vi "Save TS DAC Configuration.vi"(8 "error in":errorcluster, 11 "Generic Test Stand in":refnum<class "Generic Test Stand.lvclass">) -> (0 "error out":errorcluster, 3 "Generic Test Stand out":refnum<class "Generic Test Stand.lvclass">)   [LabVIEW 2019, in "Generic Test Stand.lvclass"]
uses:
  Generic Test Stand.lvclass
  Generic Test Stand.lvclass/Generic Test Stand.ctl
  DAC/DAC.lvclass
  <vilib>/Utility/config.llb/NI_LVConfig.lvlib
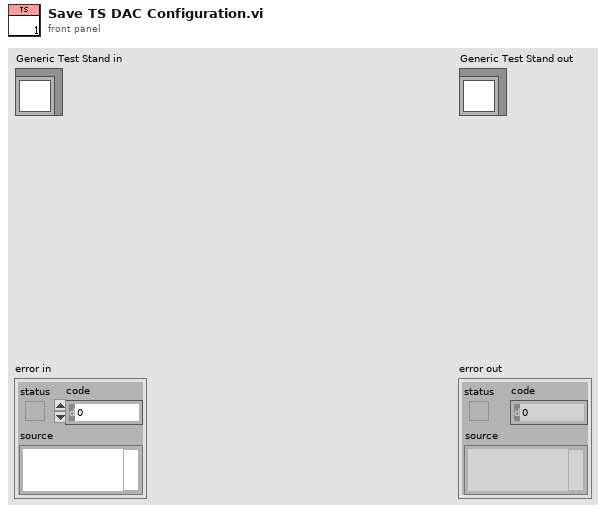
[diagram p1: front panel]
types:
  T1 = typedef "NI_LVConfig.lvlib/Config Data RefNum.ctl" = refnum<k1>
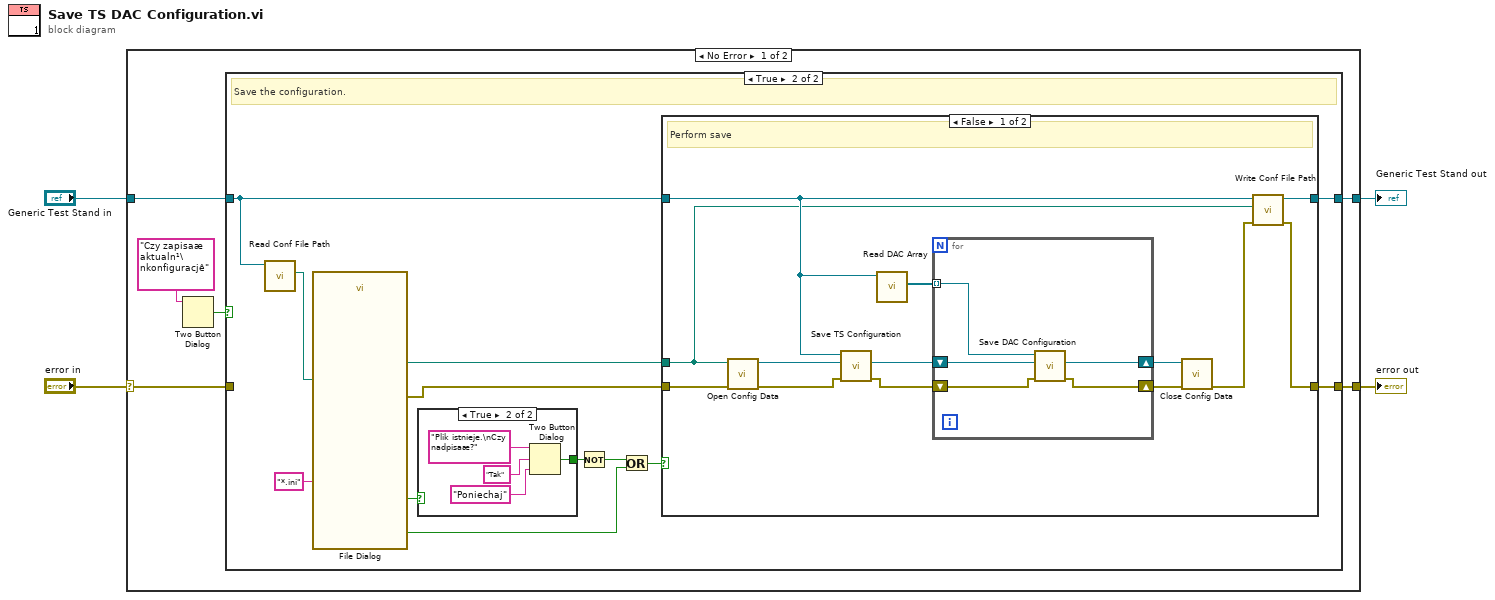
[diagram p0: block diagram]
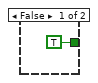
[diagram p3: hidden frame]
diagram:
  n1 = case shown="No Error" "error in" {
    selector: "error in" -> [w5 w51]
    tunnel: [w6 w51] -> w3
    tunnel: [w7 w50] -> w1
    tunnel: "Generic Test Stand in" -> [w8 w50]
    frame No Error {
      n2 = Two Button Dialog(message="Czy zapisaæ aktualn¹\nkonfiguracjê") -> (T button?=w10:bool)  [unwired: 2 in]
      n3 = case shown="True" w10 {
        tunnel: w8 -> [w12 w15]
        tunnel: [w12 w16] -> w7
        tunnel: [w11 w13] -> w6
        tunnel: w5 -> [w11 _]
        frame False {
          # "Save aborted."
        }
        frame True {
          # "Save the configuration."
          n4 = call "Read Conf File Path.vi"("Generic Test Stand in"=w15) -> ("Conf File Path"=w14:path)  [unwired: 8 in, 2 out]
          n5 = call "File Dialog"("start path"=w14, "pattern (all files)"="*.ini") -> ("selected path"=w24:path, "exists"=w21:bool, "cancelled"=w17:bool, "error out"=w23:errorcluster)  [unwired: 10 in]
          n6 = case shown="True" w21 {
            tunnel: [TRUE ("T button?") w26] -> w20
            frame False {
            }
            frame True {
              n7 = Two Button Dialog(message="Plik istnieje.\nCzy nadpisaæ?", 1:"Poniechaj" ("F button name (\"Cancel\")"), 2:"Tak" ("T button name (\"OK\")")) -> (T button?=w26:bool)
            }
          }
          n8 = Not(x=w20) -> (.not. x?=w18:bool)
          n9 = Or(x=w18, y=w17) -> (x .or. y?=w19:bool)
          n10 = case shown="False" w19 {
            tunnel: [w32 w48] -> w13
            tunnel: w24 -> [w30 _]
            tunnel: w23 -> [w42 w48]
            tunnel: w15 -> [w33 w49]
            tunnel: [w34 w49] -> w16
            frame False {
              # "Perform save"
              n11 = call <vilib>:"Open Config Data.vi"("error in (no error)"=w42, "configuration file path"=w30) -> ("error out"=w38:errorcluster, "refnum"=w36:T1)  [unwired: 7 in, 1 out]
              n12 = call-dynamic "Save TS Configuration.vi"("error in"=w38, "Config File refnum in"=w36, "Generic Test Stand in"=w33) -> ("error out"=w37:errorcluster, "Config File refnum out"=w35:T1)  [unwired: 6 in, 1 out]
              n13 = call "Read DAC Array.vi"("Generic Test Stand in"=w33) -> ("DAC Array"=w41:refnum<class "DAC.lvclass">[])  [unwired: 8 in, 2 out]
              n14 = for {
                tunnel: w41 -> [w47] mode=indexing
                shift-right: [w45] -> w40
                shift-left: w35 -> [w46]
                shift-right: [w43] -> w39
                shift-left: w37 -> [w44]
                n15 = call-dynamic "Save DAC Configuration.vi"("error in"=w44, "Config File refnum in"=w46, "DAC in"=w47) -> ("error out"=w43:errorcluster, "Config File refnum out"=w45:T1)  [unwired: 6 in, 1 out]
              }
              n16 = call <vilib>:"Close Config Data.vi"("error in (no error)"=w39, "refnum"=w40) -> ("error out"=w31:errorcluster)  [unwired: 8 in, 1 out]
              n17 = call "Write Conf File Path.vi"("error in"=w31, "Conf File Path"=w30, "Generic Test Stand in"=w33) -> ("error out"=w32:errorcluster, "Generic Test Stand out"=w34:refnum<class "Generic Test Stand.lvclass">)  [unwired: 7 in]
            }
            frame True {
              # "Save cancelled"
            }
          }
        }
      }
    }
    frame Error {
    }
  }
  "error out" <- w3
  "Generic Test Stand out" <- w1
